vi "Classify Battery.vi"(0 "Measurement":T2, 11 "error in":errorcluster) -> (4 "Chemistry":T1(ring), 6 "Charge (%)":dbl, 8 "Description":string, 15 "error out":errorcluster)   [LabVIEW 2026]
doc: "Classifies an AA cell from its Measurement by the rules of the spec, first matching rule wins: |OCV| < 0.20 V No Battery; OCV <= -0.20 V Reversed Polarity; OCV > 1.80 V Unknown; 1.40..1.60 V with Ripple pp >= 0.003 V or IR >= 1.5 Ohm Li-ion 1.5V (BMS); OCV < 1.00 V Depleted; OCV >= 1.50 V Alkaline; otherwise IR <= 0.28 Ohm Ni-MH, IR >= 0.35 Ohm Alkaline, else (IR NaN or in between) Alkaline or Ni-MH. An OCV of NaN is classified Unknown. Charge comes from Estimate Charge.vi: the chemistry's estimate, the lower of the Alkaline and Ni-MH estimates when ambiguous, 0 for Depleted, NaN otherwise. Description (Format Battery Description.vi) is one readable line naming both estimates in the ambiguous case; NaN values print as n/a. All thresholds are diagram constants of this VI; calibrated on real cells 2026-11-20 (ripple 3 mV, Ni-MH IR 0.28 Ohm), the alkaline IR limit is provisional. Pure function: error in is chained through the subVI calls to error out."
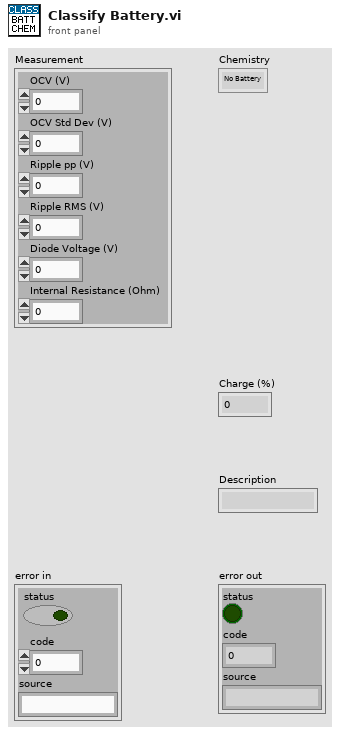
[diagram p1: front panel]
types:
  T1 = enum16{"No Battery", "Reversed Polarity", "Alkaline", "Ni-MH", "Alkaline or Ni-MH", "Li-ion 1.5V (BMS)", "Depleted", "Unknown"}
  T2 = cluster{"OCV (V)":dbl, "OCV Std Dev (V)":dbl, "Ripple pp (V)":dbl, "Ripple RMS (V)":dbl, "Diode Voltage (V)":dbl, "Internal Resistance (Ohm)":dbl}
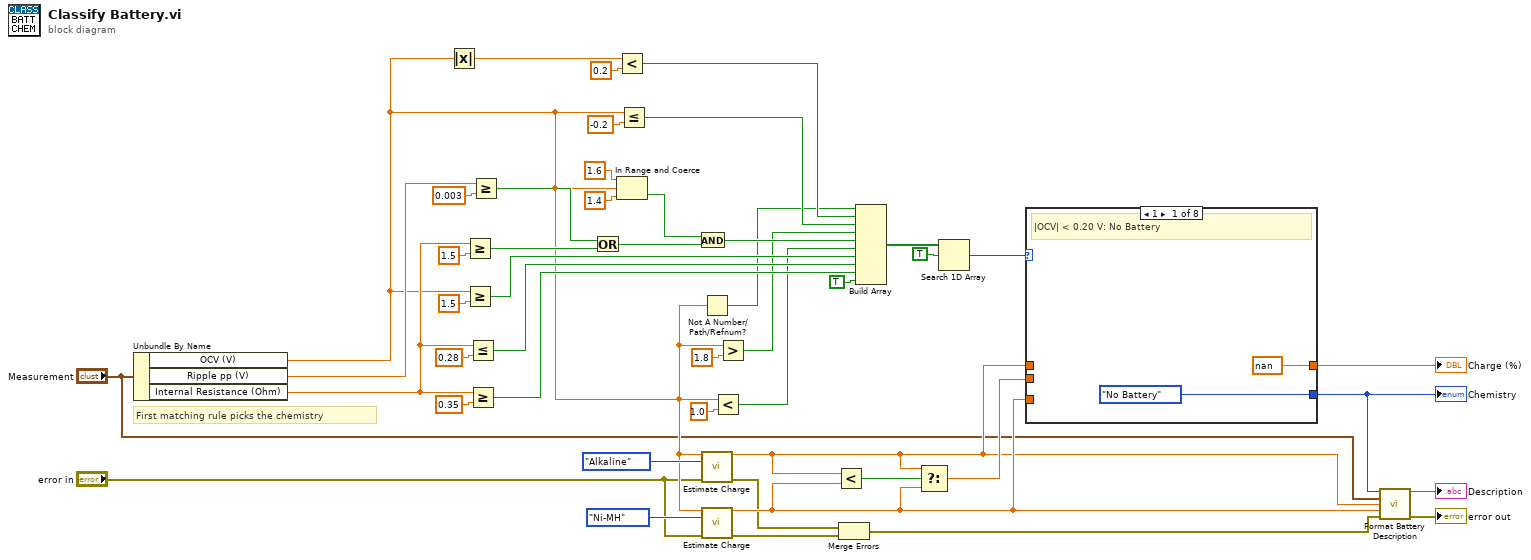
[diagram p0: block diagram]
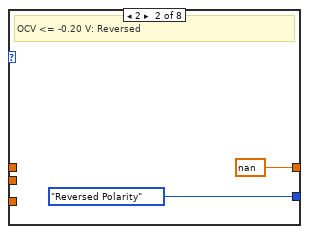
[diagram p2: hidden frame]
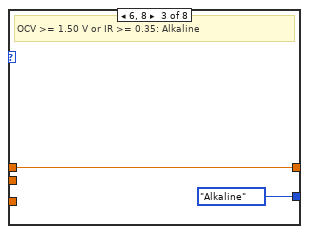
[diagram p3: hidden frame]
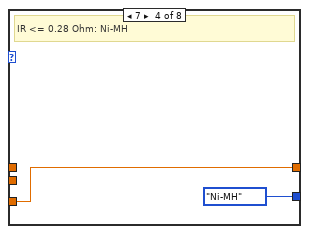
[diagram p4: hidden frame]
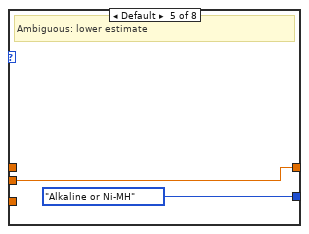
[diagram p5: hidden frame]
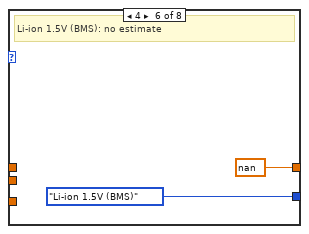
[diagram p6: hidden frame]
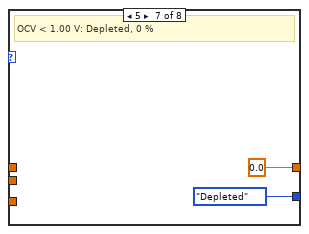
[diagram p7: hidden frame]
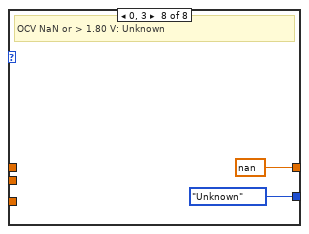
[diagram p8: hidden frame]
diagram:
  # "First matching rule picks the chemistry"
  n1 = Unbundle By Name("Measurement") -> ("OCV (V)"=w3:dbl, "Ripple pp (V)"=w4:dbl, "Internal Resistance (Ohm)"=w5:dbl)
  n2 = Absolute Value(x=w3) -> (abs(x)=w7:dbl)
  n3 = Greater Or Equal?(x=w5, y=1.5 ("Li-ion IR min (Ohm)")) -> (x >= y?=w20:bool)
  n4 = Greater Or Equal?(x=w3, y=1.5 ("alkaline at or above (V)")) -> (x >= y?=w26:bool)
  n5 = Less Or Equal?(x=w5, y=0.28 ("Ni-MH IR max (Ohm)")) -> (x <= y?=w28:bool)
  n6 = Greater Or Equal?(x=w5, y=0.35 ("alkaline IR min (Ohm)")) -> (x >= y?=w30:bool)
  n7 = Greater Or Equal?(x=w4, y=0.003 ("Li-ion ripple min (V)")) -> (x >= y?=w18:bool)
  n8 = Or(x=w18, y=w20) -> (x .or. y?=w21:bool)
  n9 = Less?(x=w7, y=0.2 ("no battery below (V)")) -> (x < y?=w9:bool)
  n10 = In Range and Coerce(upper limit=1.6 ("Li-ion window high (V)"), x=w3, lower limit=1.4 ("Li-ion window low (V)")) -> (In Range?=w16:bool)  [unwired: 1 out]
  n11 = Less Or Equal?(x=w3, y=-0.2 ("reversed at or below (V)")) -> (x <= y?=w11:bool)
  n12 = And(x=w16, y=w21) -> (x .and. y?=w22:bool)
  n13 = Not A Number/Path/Refnum?(number/path/refnum=w3) -> (NaN/Path/Refnum?=w6:bool)
  n14 = call "Estimate Charge.vi"("OCV (V)"=w3, "Chemistry"=T1."Alkaline" ("Alkaline"), "error in"="error in") -> ("Charge (%)"=w36:dbl, "error out"=w37:errorcluster)  [unwired: 11 in]
  n15 = call "Estimate Charge.vi"("OCV (V)"=w3, "Chemistry"=T1."Ni-MH" ("Ni-MH"), "error in"="error in") -> ("Charge (%)"=w39:dbl, "error out"=w40:errorcluster)  [unwired: 11 in]
  n16 = Less?(x=w3, y=1.0 ("depleted below (V)")) -> (x < y?=w24:bool)
  n17 = Greater?(x=w3, y=1.8 ("single cell max (V)")) -> (0:w13:bool)
  n18 = Less?(x=w36, y=w39) -> (x < y?=w42:bool)
  n19 = Merge Errors(w37, w40) -> (w41:errorcluster)
  n20 = Build Array(w6, w9, w11, w13, w22, w24, w26, w28, w30, TRUE ("otherwise")) -> (w32:bool[])
  n21 = Select(t=w36, s=w42, f=w39) -> (s? t:f=w43:dbl)
  n22 = Search 1D Array(1D array=w32, element=TRUE ("match")) -> (index of element=w34:i32)  [unwired: 1 in]
  n23 = case shown="1" w34 {
    tunnel: [nan ("charge") nan ("charge") w52 w54 w56 nan ("charge") 0.0 ("charge") nan ("charge")] -> w44
    tunnel: [T1."No Battery" ("chemistry") T1."Reversed Polarity" ("chemistry") T1."Alkaline" ("chemistry") T1."Ni-MH" ("chemistry") T1."Alkaline or Ni-MH" ("chemistry") T1."Li-ion 1.5V (BMS)" ("chemistry") T1."Depleted" ("chemistry") T1."Unknown" ("chemistry")] -> w45
    tunnel: w36 -> [_ _ w52 _ _ _ _ _]
    tunnel: w39 -> [_ _ _ w54 _ _ _ _]
    tunnel: w43 -> [_ _ _ _ w56 _ _ _]
    frame 1 {
      # "|OCV| < 0.20 V: No Battery"
    }
    frame 2 {
      # "OCV <= -0.20 V: Reversed"
    }
    frame 6, 8 {
      # "OCV >= 1.50 V or IR >= 0.35: Alkaline"
    }
    frame 7 {
      # "IR <= 0.28 Ohm: Ni-MH"
    }
    frame Default {
      # "Ambiguous: lower estimate"
    }
    frame 4 {
      # "Li-ion 1.5V (BMS): no estimate"
    }
    frame 5 {
      # "OCV < 1.00 V: Depleted, 0 %"
    }
    frame 0, 3 {
      # "OCV NaN or > 1.80 V: Unknown"
    }
  }
  "Chemistry" <- w45
  "Charge (%)" <- w44
  n24 = call "Format Battery Description.vi"("Chemistry"=w45, "Measurement"="Measurement", "Alkaline Charge (%)"=w36, "Ni-MH Charge (%)"=w39, "error in"=w41) -> ("Description"=→"Description":string, "error out"=→"error out":errorcluster)  [unwired: 9 in]
